vi "SDO_TRAJ_CALC_ORIENTATION.vi"(0 "Total Trajectory Time":dbl, 4 "Starting Fraction":dbl=0.1, 6 "Completion Fraction":dbl=0.8, 8 "Init":bool, 9 "Time Fraction":dbl, 10 "End Orientation Demand DEG":dbl, 11 "Starting Orientation  DEG":dbl) -> (1 "Rotational Velocity":dbl, 2 "Orientation Demand Deg":dbl, 3 "Orientation Demand":T1 {"SIN" format="%13.4f"; "COS" format="%13.4f"; "VALUE" format="%13.4f"})   [LabVIEW 2019]
uses:
  <vilib>/Rock Robotics/WPI/ThirdParty/JAS_Junk/TrajLib/TypeDef/ROTATION2D.ctl
  <vilib>/Rock Robotics/WPI/ThirdParty/JAS_Junk/TrajLib/Conv_Deg_Radians.vi
  <vilib>/Rock Robotics/WPI/ThirdParty/JAS_Junk/TrajLib/Rotation2d_CreateAngle.vi
  <vilib>/Rock Robotics/WPI/ThirdParty/JAS_Junk/TrajLib/Rotation2d_Plus.vi
  <vilib>/Rock Robotics/WPI/ThirdParty/JAS_Junk/TrajLib/MathUtil_Clamp.vi
  <vilib>/Rock Robotics/WPI/ThirdParty/JAS_Junk/TrajLib/Rotation2d_Times.vi
  <vilib>/Rock Robotics/WPI/ThirdParty/JAS_Junk/TrajLib/Rotation2d_UnaryMinus.vi
  <vilib>/Rock Robotics/WPI/ThirdParty/JAS_Junk/TrajLib/Rotation2d_RotateBy.vi
  <vilib>/Rock Robotics/WPI/ThirdParty/JAS_Junk/TrajLib/Conv_Radians_Deg.vi
  <vilib>/Rock Robotics/WPI/ThirdParty/JAS_Junk/TrajLib/Rotation2d_CreateXY.vi
  <vilib>/Rock Robotics/WPI/ThirdParty/JAS_Junk/TrajLib/Util_CalcDist.vi
  <vilib>/Rock Robotics/WPI/ThirdParty/JAS_Junk/TrajLib/Trajectory_Library.lvlib
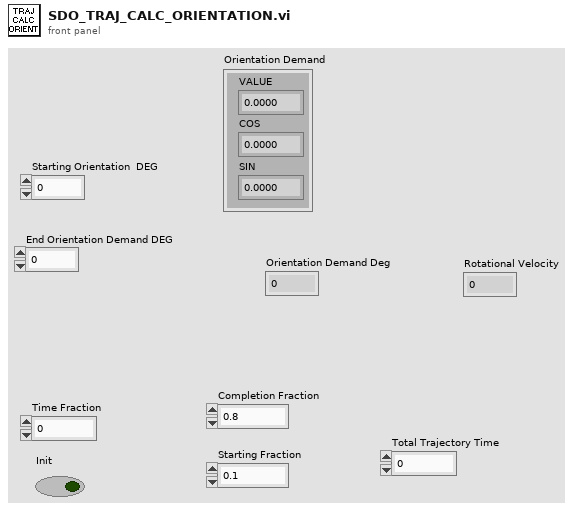
[diagram p1: front panel]
types:
  T1 = typedef "Trajectory_Library.lvlib/ROTATION2D.ctl" = cluster{"VALUE":dbl, "COS":dbl, "SIN":dbl}
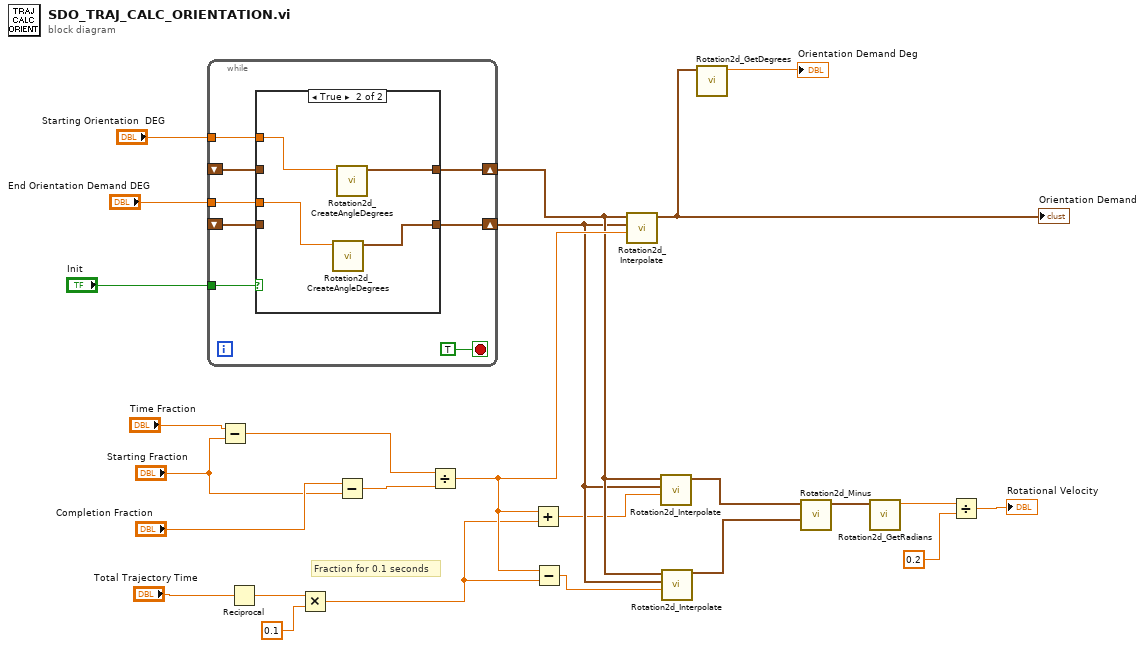
[diagram p0: block diagram]
diagram:
  # "Fraction for 0.1 seconds"
  n1 = while {
    tunnel: "Init" -> [w32]
    tunnel: "End Orientation Demand DEG" -> [w31]
    shift-right: [w29] -> w8
    shift-left: _ -> [w27]
    shift-right: [w30] -> w9
    shift-left: _ -> [w28]
    tunnel: "Starting Orientation  DEG" -> [w26]
    stop <- TRUE stop-if-true
    n2 = case shown="True" w32 {
      tunnel: w31 -> [_ w39]
      tunnel: [w35 w36] -> w30
      tunnel: [w34 w38] -> w29
      tunnel: w28 -> [w35 _]
      tunnel: w27 -> [w34 _]
      tunnel: w26 -> [_ w37]
      frame False {
      }
      frame True {
        n3 = call <vilib>:"Rotation2d_CreateAngleDegrees.vi"("Angle_Degrees"=w39) -> ("ROTATION"=w38:T1)  [unwired: 10 in]
        n4 = call <vilib>:"Rotation2d_CreateAngleDegrees.vi"("Angle_Degrees"=w37) -> ("ROTATION"=w36:T1)  [unwired: 10 in]
      }
    }
  }
  n5 = Subtract(x="Time Fraction", y="Starting Fraction") -> (x-y=w19:dbl)
  n6 = Reciprocal(x="Total Trajectory Time") -> (1/x=w13:dbl)
  n7 = Multiply(x=w13, y=0.1) -> (x*y=w10:dbl)
  n8 = Subtract(x="Completion Fraction", y="Starting Fraction") -> (x-y=w20:dbl)
  n9 = Divide(x=w19, y=w20) -> (x/y=w11:dbl)
  n10 = Add(x=w11, y=w10) -> (x+y=w7:dbl)
  n11 = Subtract(x=w11, y=w10) -> (x-y=w6:dbl)
  n12 = call <vilib>:"Rotation2d_Interpolate.vi"("T"=w11, "EncValue ROTATION"=w8, "in ROTATION"=w9) -> ("Interpolated ROTATION"=w17:T1)  [unwired: 8 in]
  "Orientation Demand" <- w17
  n13 = call <vilib>:"Rotation2d_Interpolate.vi"("T"=w7, "EncValue ROTATION"=w8, "in ROTATION"=w9) -> ("Interpolated ROTATION"=w5:T1)  [unwired: 8 in]
  n14 = call <vilib>:"Rotation2d_Interpolate.vi"("T"=w6, "EncValue ROTATION"=w8, "in ROTATION"=w9) -> ("Interpolated ROTATION"=w4:T1)  [unwired: 8 in]
  n15 = call <vilib>:"Rotation2d_GetDegrees.vi"("in ROTATION"=w17) -> ("AngleDegrees"=→"Orientation Demand Deg":dbl)  [unwired: 10 in]
  n16 = call <vilib>:"Rotation2d_Minus.vi"("other ROTATION"=w4, "in ROTATION"=w5) -> ("out ROTATION"=w3:T1)  [unwired: 9 in]
  n17 = call <vilib>:"Rotation2d_GetRadians.vi"("in ROTATION"=w3) -> ("AngleRadians"=w2:dbl)  [unwired: 10 in]
  n18 = Divide(x=w2, y=0.2) -> (x/y=→"Rotational Velocity":dbl)
